vi "05a-multiple_functions.vi"() -> ()   [LabVIEW 2018, in "LV2Julia_examples.lvlib"]
uses:
  LV2Julia_examples.lvlib
  LV2Julia_core/VIs/Server or client state.ctl
  LV2Julia_core/VIs/detailed error info.ctl
  LV2Julia_core/VIs/StackFrame.ctl
  LV2Julia_core/VIs/Commands.ctl
  1e32e5d8-80f1-4661-9552-ce4369739336.vi
  1e32e5d8-80f1-4661-9552-ce4369739336.vi/97f15dbd-49bd-450f-b5c2-f596e30d06e1.vi
  1e32e5d8-80f1-4661-9552-ce4369739336.vi/97f15dbd-49bd-450f-b5c2-f596e30d06e1.vi/51a7904d-5826-47e1-a1e5-6a2c4d0d0a4a.vi
  1e32e5d8-80f1-4661-9552-ce4369739336.vi/97f15dbd-49bd-450f-b5c2-f596e30d06e1.vi/1ddba192-2c06-4eed-b8c8-4b8dd3e91ecf.vi
  1e32e5d8-80f1-4661-9552-ce4369739336.vi/97f15dbd-49bd-450f-b5c2-f596e30d06e1.vi/eb296ac8-068e-4c2a-b767-f4fb9983b002.vi
  LV2Julia_core/VIs/jl-scripts path.vi
  LV2Julia_core/VIs/check ID validity.vi
  LV2Julia_core/VIs/bindata_descr to JSON.vi
  LV2Julia_core/VIs/check cluster field names.vi
  LV2Julia_core/VIs/concat JSON.vi
  LV2Julia_core/VIs/build request.vi
  LV2Julia_core/VIs/Parse server response.vi
  LV2Julia_core/VIs/log jl exceptions.vi
  LV2Julia_core/LV2Julia_core.lvlib
panel:
  in  "operation":T1(radio)
  in  "operands":cluster{"x":dbl, "y":dbl}={"x"=2.0, "y"=2.0}
  in  "next":bool
  out "x OP y":dbl=nan
  out "detailed error info":T2
  out "current error":errorcluster
  out "final error":errorcluster
  out "short err code":u8
  in  "stop":bool
  out "ZMQ timeout":bool
  out "Julia script file path":path
  out "temporary script path":path
  out "Jl Server state":T4
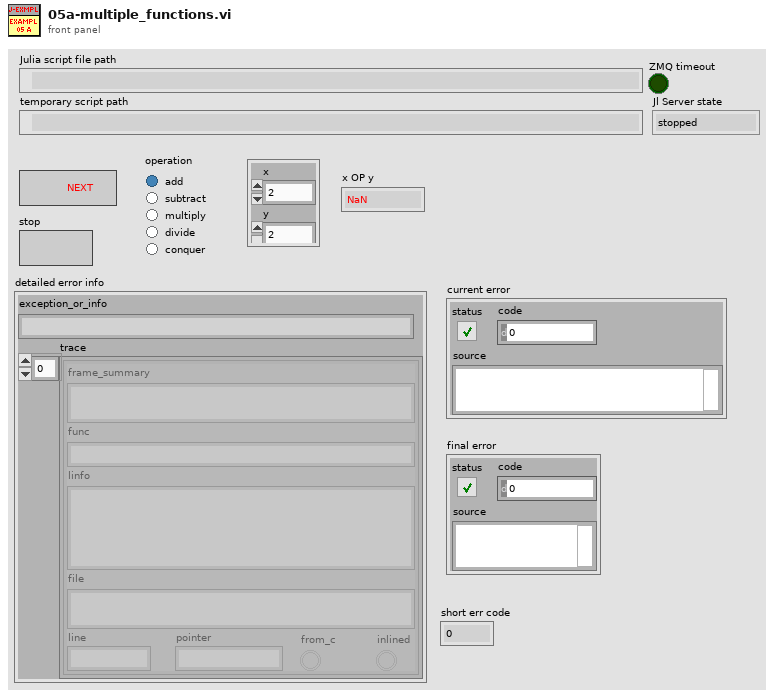
[diagram p1: front panel]
types:
  T1 = enum32{"add", "subtract", "multiply", "divide", "conquer"}
  T2 = typedef "LV2Julia_core.lvlib/detailed error info.ctl" = cluster{"exception_or_info":string, "trace":T3[]}
  T3 = typedef "LV2Julia_core.lvlib/StackFrame.ctl" = cluster{"frame_summary":string, "func":string, "linfo":string, "file":string, "line":i32, "pointer":u64, "from_c":bool, "inlined":bool}
  T4 = typedef "LV2Julia_core.lvlib/Server or client state.ctl" = enum16{"stopped", "running", "unknown"}
  T5 = typedef "LV2Julia_core.lvlib/Commands.ctl" = enum16{"Start Jl-server & Init LV-client", "Send request & Get response ", "Stop Jl-server & Cleanup LV-client", "Cleanup LV-client", "Start Jl-server", "Stop Jl-server", "Init LV-Client", "Cleanup LV-Client", "(not allowed)", "Set LV Client state", "Set Jl Server state", "set ZMQ timeout", "read ZMQ timeout", "read-out state"}
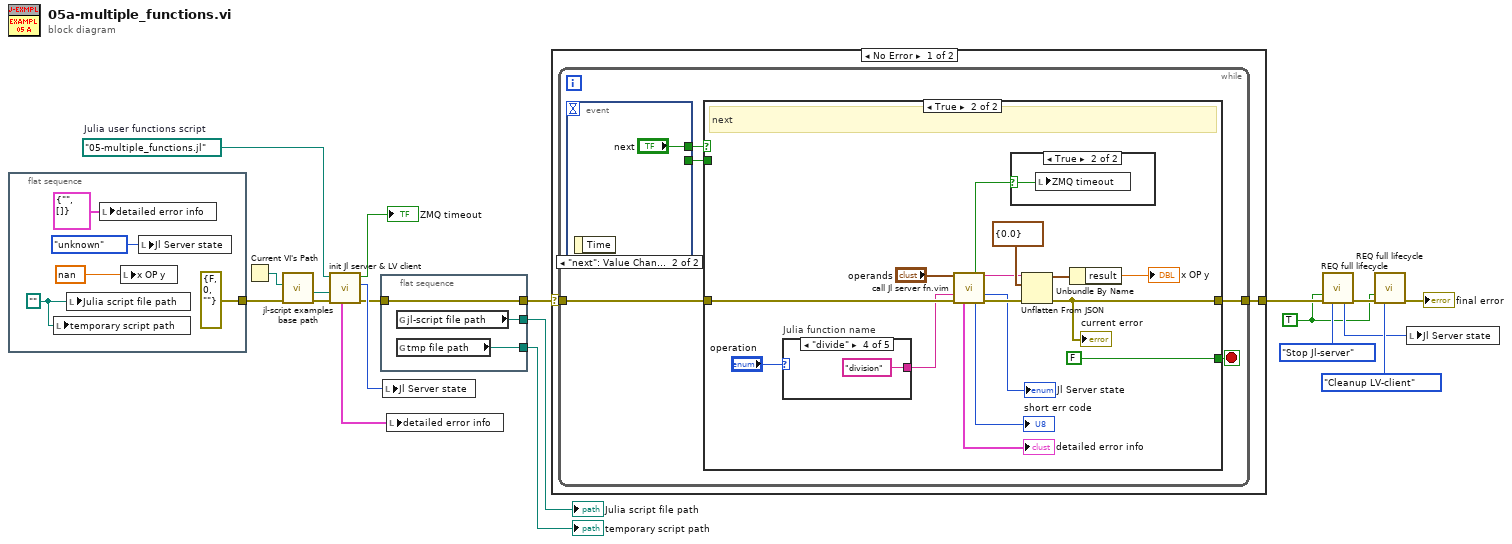
[diagram p0: block diagram]
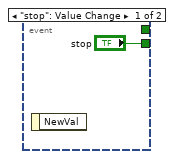
[diagram p2: hidden frame]
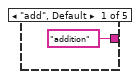
[diagram p4: hidden frame]
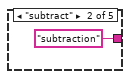
[diagram p5: hidden frame]
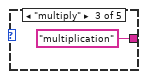
[diagram p6: hidden frame]
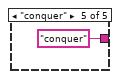
[diagram p7: hidden frame]
diagram:
  w9 = path "05-multiple_functions.jl"  # Julia user functions script
  w10 = TRUE ("Force command")
  n1 = flat-sequence {
    tunnel: [errorcluster {"status"=FALSE, "code"=0, "source"=""} ("error in (no error)")] -> w2
    frame #0 {
      w20 = path ""
      n2 = local write "temporary script path"(w20) -> ()
      n3 = local write "Julia script file path"(w20) -> ()
      n4 = local write "detailed error info"(T2 {"exception_or_info"="", "trace"=[]} ("detailed error info")) -> ()
      n5 = local write "x OP y"(nan ("Server response")) -> ()
      n6 = local write "Jl Server state"(Server_or_client_state."unknown" ("Jl Server state out")) -> ()
    }
  }
  n7 = Current VI's Path() -> (path=w5:path)
  n8 = call "jl-script examples base path.vi"("error in (no error)"=w2, "calling example VI path"=w5) -> ("error out"=w4:errorcluster, "jl-script-examples base path"=w3:path)  [unwired: 8 in]
  n9 = call "init Jl server & LV client.vi"("error in (no error)"=w4, "Base path (not a path)"=w3, "Julia user functions script"=w9) -> ("error out"=w6:errorcluster, "Jl Server state out"=w8:T4, "timeout?"=→"ZMQ timeout":bool, "detailed error info"=w1:T2)  [unwired: 3 in, 2 out]
  n10 = flat-sequence {
    tunnel: [w27] -> w14
    tunnel: w6 -> [w27]
    tunnel: [w26] -> w12
    tunnel: [w25] -> w13
    frame #0 {
      n11 = global read "jl-scripts path.vi" "jl-script file path"() -> (w26:path)
      n12 = global read "jl-scripts path.vi" "tmp file path"() -> (w25:path)
    }
  }
  n13 = local write "Jl Server state"(w8) -> ()
  n14 = local write "detailed error info"(w1) -> ()
  n15 = case shown="No Error" w14 {
    selector: w14 -> [w28 w60]
    tunnel: [w29 w60] -> w19
    frame No Error {
      n16 = while {
        tunnel: w28 -> [w33]
        tunnel: [w34] -> w29
        stop <- w31 stop-if-true
        n17 = event shown="[1] \"next\": Value Change" {
          selector: _ -> [_ _]
          dyn-events: _ -> [_ _]
          timeout: _ -> [_ _]
          tunnel: [_ "next"] -> w32
          tunnel: ["stop" _] -> w30
          event "stop": Value Change {
            n18 = event-data() -> ()  [unwired: 1 in, 1 out]
          }
          event "next": Value Change {
            n19 = event-data() -> ()  [unwired: 1 in, 1 out]
          }
        }
        n20 = case shown="True" w32 {
          tunnel: [w38 w50] -> w34
          tunnel: w33 -> [w38 w46]
          tunnel: [w37 FALSE ("stop this VI only")] -> w31
          tunnel: w30 -> [w37 _]
          frame False {
            # "stop"
          }
          frame True {
            # "next"
            n21 = case "Julia function name" shown="\"divide\"" "operation" {
              tunnel: ["addition" "subtraction" "multiplication" "division" "conquer"] -> w45
              frame "add", Default {
              }
              frame "subtract" {
              }
              frame "multiply" {
              }
              frame "divide" {
              }
              frame "conquer" {
              }
            }
            n22 = call "call Jl server fn.vim"("Arguments 1"="operands", "fun2call"=w45, "error in (no error)"=w46) -> ("timeout?"=w42:bool, "JSON received"=w41:string, "Jl Server state out"=→"Jl Server state":T4, "detailed error info"=→"detailed error info":T2, "return code"=→"short err code":u8, "error out"=w47:errorcluster)  [unwired: 6 in, 1 out]
            n23 = case shown="True" w42 {
              selector: w42 -> [_ w59]
              frame False {
              }
              frame True {
                n24 = local write "ZMQ timeout"(w59) -> ()
              }
            }
            n25 = Unflatten From JSON(JSON string=w41, type and defaults=cluster{"result":dbl} {"result"=0.0} ("parsed response"), error in (no error)=w47) -> (value=w52:cluster{"result":dbl}, error out=w50:errorcluster)  [unwired: 4 in]
            "current error" <- w50
            n26 = Unbundle By Name(w52) -> ("result"=→"x OP y":dbl)
          }
        }
      }
    }
    frame Error {
    }
  }
  n27 = call "REQ full lifecycle.vi"("Force command"=w10, "error in"=w19, "command"=Commands."Stop Jl-server") -> ("Jl Server state out"=w11:T4, "error out"=w17:errorcluster)  [unwired: 6 in, 5 out]
  n28 = call "REQ full lifecycle.vi"("Force command"=w10, "error in"=w17, "command"=Commands."Cleanup LV-client") -> ("error out"=→"final error":errorcluster)  [unwired: 6 in, 6 out]
  n29 = local write "Jl Server state"(w11) -> ()
  "temporary script path" <- w13
  "Julia script file path" <- w12
